vi "LinearFilter_Calculate.vi"(9 "Input":dbl format="%13.5p", 11 "In LINEAR_FILTER":T1 {"Outputs" format="%13.5g"; "Inputs" format="%13.5g"; "OutputGains" format="%13.5g"; "InputGains" format="%13.5g"}) -> (1 "Output":dbl format="%13.5p", 3 "Out LINEAR_FILTER":T1 {"Outputs" format="%13.5g"; "Inputs" format="%13.5g"; "OutputGains" format="%13.5g"; "InputGains" format="%13.5g"})   [LabVIEW 2019, in "Trajectory_Library.lvlib"]
doc: "Calculates the next value of the filter. To work correctly this must be called periodically\n\nInputs:\n - inLinearfilter - Linear filter data structure\n - input - Current input value.\n \nOutputs:\n - outLinearfilter - Updated linear filter data structurea\n - output - The filtered value at this step"
uses:
  Trajectory_Library.lvlib
  TypeDef/LINEAR_FILTER.ctl
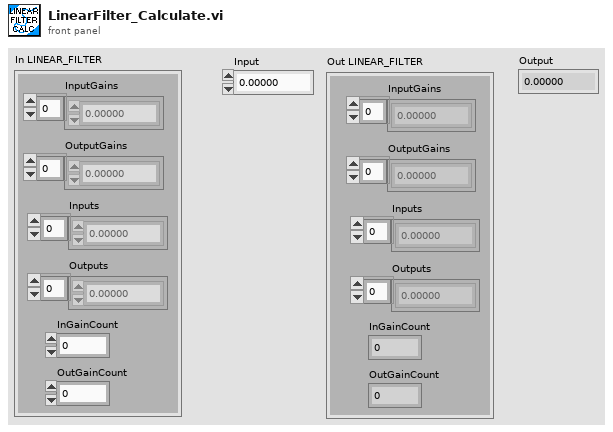
[diagram p1: front panel]
types:
  T1 = typedef "Trajectory_Library.lvlib/LINEAR_FILTER.ctl" = cluster{"InputGains":dbl[], "OutputGains":dbl[], "Inputs":dbl[], "Outputs":dbl[], "InGainCount":i32, "OutGainCount":i32}
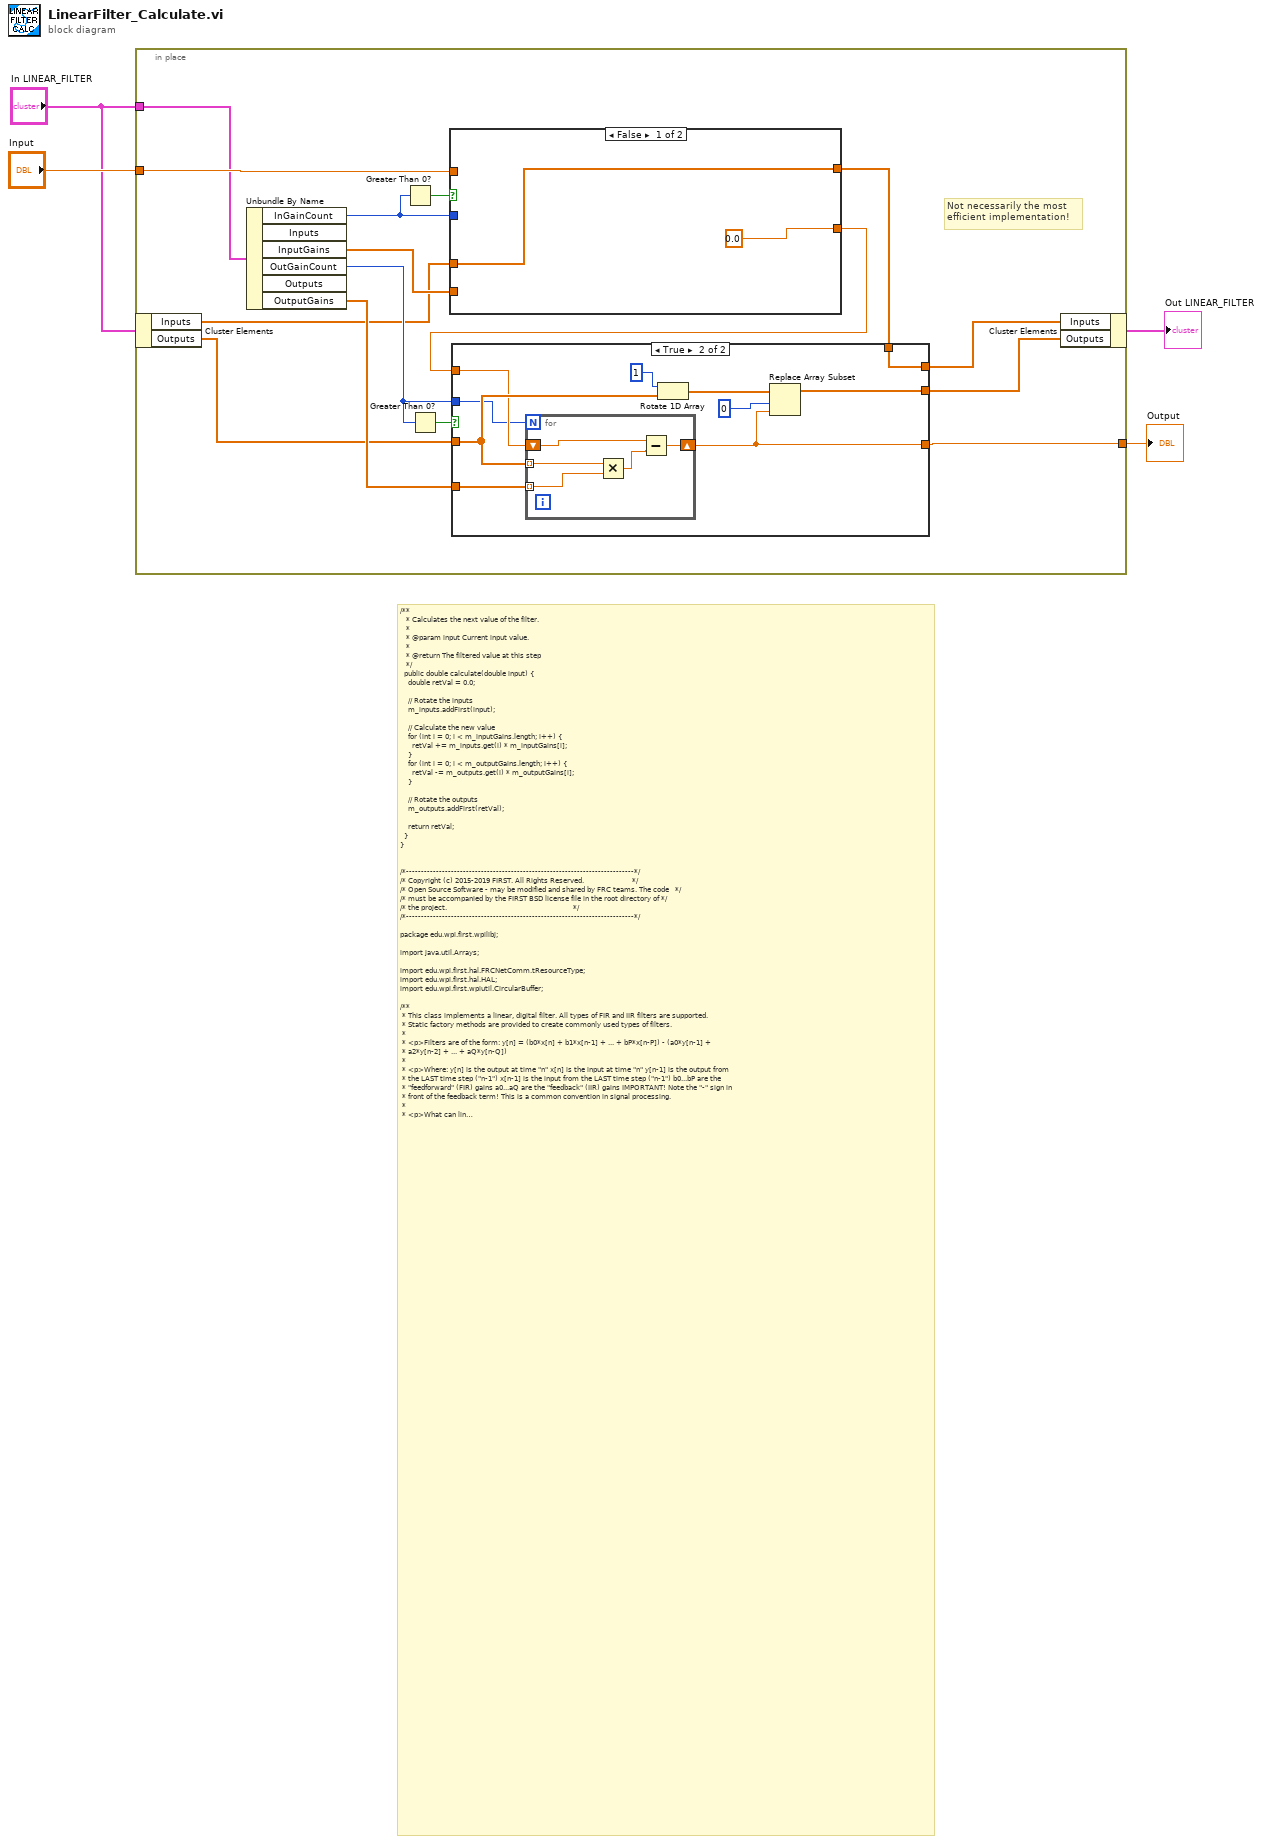
[diagram p0: block diagram]
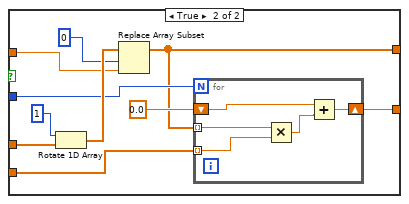
[diagram p3: hidden frame]
diagram:
  # "/**\n   * Calculates the next value of the filter.\n   *\n   * @param input Current input value.\n   *\n   * @return The filtered value at this step\n   */\n  public double calculate(double input) {\n    double retVal = 0.0;\n\n    // Rotate the inputs\n    m_inputs.addFirst(input);\n\n    // Calculate the new value\n    for (int i = 0; i < m_inputGains.length; i++) {\n      retVal += m_inputs.get(i) * m_inputGains[i];\n    }\n    for (int i = 0; i < m_outputGains.length; i++) {\n      retVal -= m_outputs.get(i) * m_outputGains[i];\n    }\n\n    // Rotate the outputs\n    m_outputs.addFirst(retVal);\n\n    return retVal;\n  }\n}\n\n\n/*----------------------------------------------------------------------------*/\n/* Copyright (c) 2015-2019 FIRST. All Rights Reserved.                        */\n/* Open Source Software - may be modified and shared by FRC teams. The code   */\n/* must be accompanied by the FIRST BSD license file in the root directory of */\n/* the project.                                                               */\n/*----------------------------------------------------------------------------*/\n\npackage edu.wpi.first.wpilibj;\n\nimport java.util.Arrays;\n\nimport edu.wpi.first.hal.FRCNetComm.tResourceType;\nimport edu.wpi.first.hal.HAL;\nimport edu.wpi.first.wpiutil.CircularBuffer;\n\n/**\n * This class implements a linear, digital filter. All types of FIR and IIR filters are supported.\n * Static factory methods are provided to create commonly used types of filters.\n *\n * <p>Filters are of the form: y[n] = (b0*x[n] + b1*x[n-1] + ... + bP*x[n-P]) - (a0*y[n-1] +\n * a2*y[n-2] + ... + aQ*y[n-Q])\n *\n * <p>Where: y[n] is the output at time \"n\" x[n] is the input at time \"n\" y[n-1] is the output from\n * the LAST time step (\"n-1\") x[n-1] is the input from the LAST time step (\"n-1\") b0...bP are the\n * \"feedforward\" (FIR) gains a0...aQ are the \"feedback\" (IIR) gains IMPORTANT! Note the \"-\" sign in\n * front of the feedback term! This is a common convention in signal processing.\n *\n * <p>What can linear filters do? Basically, they can filter, or diminish, the effects of\n * undesirable input frequencies. High frequencies, or rapid changes, can be indicative of sensor\n * noise or be otherwise undesirable. A \"low pass\" filter smooths out the signal, reducing the\n * impact of these high frequency components.  Likewise, a \"high pass\" filter gets rid of\n * slow-moving signal components, letting you detect large changes more easily.\n *\n * <p>Example FRC applications of filters: - Getting rid of noise from an analog sensor input (note:\n * the roboRIO's FPGA can do this faster in hardware) - Smoothing out joystick input to prevent the\n * wheels from slipping or the robot from tipping - Smoothing motor commands so that unnecessary\n * strain isn't put on electrical or mechanical components - If you use clever gains, you can make a\n * PID controller out of this class!\n *\n * <p>For more on filters, we highly recommend the following articles:<br>\n * https://en.wikipedia.org/wiki/Linear_filter<br>\n * https://en.wikipedia.org/wiki/Iir_filter<br>\n * https://en.wikipedia.org/wiki/Fir_filter<br>\n *\n * <p>Note 1: calculate() should be called by the user on a known, regular period. You can use a\n * Notifier for this or do it \"inline\" with code in a periodic function.\n *\n * <p>Note 2: For ALL filters, gains are necessarily a function of frequency. If you make a filter\n * that works well for you at, say, 100Hz, you will most definitely need to adjust the gains if you\n * then want to run it at 200Hz! Combining this with Note 1 - the impetus is on YOU as a developer\n * to make sure calculate() gets called at the desired, constant frequency!\n */"
  n1 = in-place {
    in-place-border: "Input" -> [w17]
    in-place-border: "In LINEAR_FILTER" -> [w14]
    in-place-border: [w12] -> w3
    # "Not necessarily the most\nefficient implementation!"
    n2 = in-place-cluster #1("In LINEAR_FILTER") -> ("Inputs"=w8:dbl[], "Outputs"=w7:dbl[])
    n3 = Unbundle By Name(w14) -> ("InGainCount"=w11:i32, "InputGains"=w16:dbl[], "OutGainCount"=w10:i32, "OutputGains"=w15:dbl[])  [unwired: 2 out]
    n4 = Greater Than 0?(x=w11) -> (x > 0?=w19:bool)
    n5 = Greater Than 0?(x=w10) -> (x > 0?=w18:bool)
    n6 = case shown="False" w19 {
      tunnel: w8 -> [w38 w49]
      tunnel: w17 -> [_ w46]
      tunnel: w16 -> [_ w42]
      tunnel: [0.0 w43] -> w13
      tunnel: w11 -> [_ w41]
      tunnel: [w38 w40] -> w5
      frame False {
      }
      frame True {
        n7 = Rotate 1D Array(1:w49, 2:1 ("n")) -> (0:w47:dbl[])
        n8 = Replace Array Subset(array=w47, new element=w46, index=0) -> (w40:dbl[])
        n9 = for {
          N: w41 -> [_]
          shift-right: [w54] -> w43
          shift-left: 0.0 -> [w53]
          tunnel: w40 -> [w51] mode=indexing
          tunnel: w42 -> [w50] mode=indexing
          n10 = Multiply(x=w51, y=w50) -> (x*y=w52:dbl)
          n11 = Add(x=w53, y=w52) -> (x+y=w54:dbl)
        }
      }
    }
    n12 = case shown="True" w18 {
      tunnel: w7 -> [w21 w28]
      tunnel: w15 -> [_ w27]
      tunnel: w13 -> [w22 w26]
      tunnel: [w22 w29] -> w12
      tunnel: w10 -> [_ w25]
      tunnel: [w21 w24] -> w9
      tunnel: [w20 w23] -> w6
      tunnel: w5 -> [w20 w23]
      frame False {
      }
      frame True {
        n13 = for {
          N: w25 -> [_]
          shift-right: [w37] -> w29
          shift-left: w26 -> [w36]
          tunnel: w28 -> [w34] mode=indexing
          tunnel: w27 -> [w33] mode=indexing
          n14 = Multiply(x=w34, y=w33) -> (x*y=w35:dbl)
          n15 = Subtract(x=w36, y=w35) -> (x-y=w37:dbl)
        }
        n16 = Rotate 1D Array(1:w28, 2:1 ("n")) -> (0:w31:dbl[])
        n17 = Replace Array Subset(array=w31, new element=w29, index=0) -> (w24:dbl[])
      }
    }
    n18 = in-place-cluster #1("Inputs"=w6, "Outputs"=w9) -> (→"Out LINEAR_FILTER":T1)
  }
  "Output" <- w3
